vi "Configure Module.vi"(8 "error in (no error)":errorcluster, 10 "IOV ref in":variant, 11 "RSI Module in":refnum<class "RSI Module.lvclass">) -> (0 "error out":errorcluster, 2 "IOV ref out":variant, 3 "RSI Module out":refnum<class "RSI Module.lvclass">)   [LabVIEW 2020, in "Modules.lvlib" / "RSI Module.lvclass"]
uses:
  RSI Module.lvclass
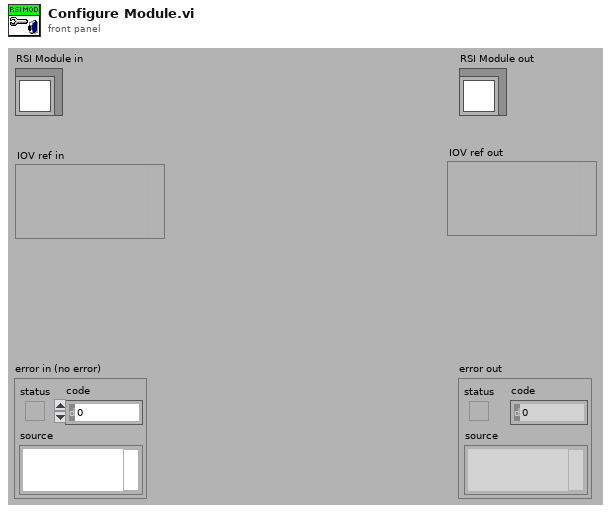
[diagram p1: front panel]
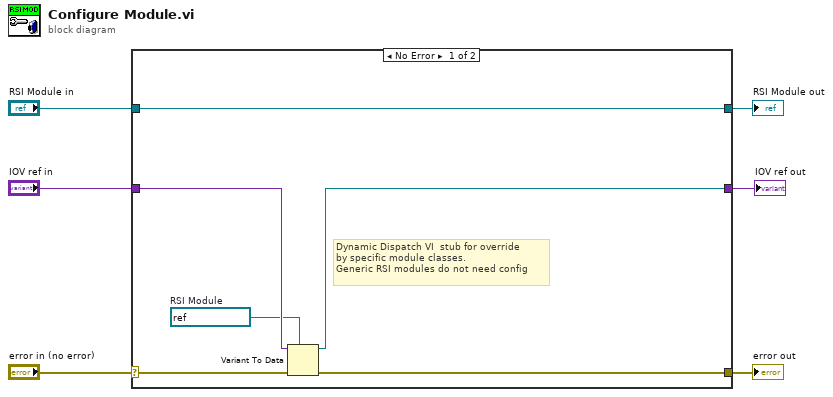
[diagram p0: block diagram]
diagram:
  n1 = case shown="No Error" "error in (no error)" {
    selector: "error in (no error)" -> [w11 w15]
    tunnel: [w10 w15] -> w5
    tunnel: [w12 w14] -> w3
    tunnel: "RSI Module in" -> [w12 w14]
    tunnel: "IOV ref in" -> [w9 w13]
    tunnel: [w8 w13] -> w1
    frame No Error {
      w7 = refnum<k21> refnum  # RSI Module
      # "Dynamic Dispatch VI  stub for override\nby specific module classes.\nGeneric RSI modules do not need config"
      n2 = Variant To Data(error in=w11, type=w7, Variant=w9) -> (data=w8:refnum<k21>, error out=w10:errorcluster)
    }
    frame Error {
    }
  }
  "error out" <- w5
  "RSI Module out" <- w3
  "IOV ref out" <- w1
